vi "RemoteVI Send Origin.vi"(0 "clients":T1(array[cluster]), 5 "origin":cluster{"x":i32, "y":i32}, 7 "origin sent":cluster{"x":i32, "y":i32}) -> (4 "clients out":T1(array[cluster]), 6 "origin sent out":cluster{"x":i32, "y":i32})   [LabVIEW 2020, in "RemoteVI.lvlib"]
doc: "Tells every client where the panel area now starts inside the frame, when that changed: if origin differs from origin sent (the origin the clients were last told - new clients get the current one with their greeting), the text message origin x y (RemoteVI Origin Message.vi) is written to every client that is not closed (RemoteVI Write To Clients.vi, 500 ms per client; a failed write marks the client closed) and origin sent out becomes origin. Otherwise nothing is written."
uses:
  RemoteVI.lvlib
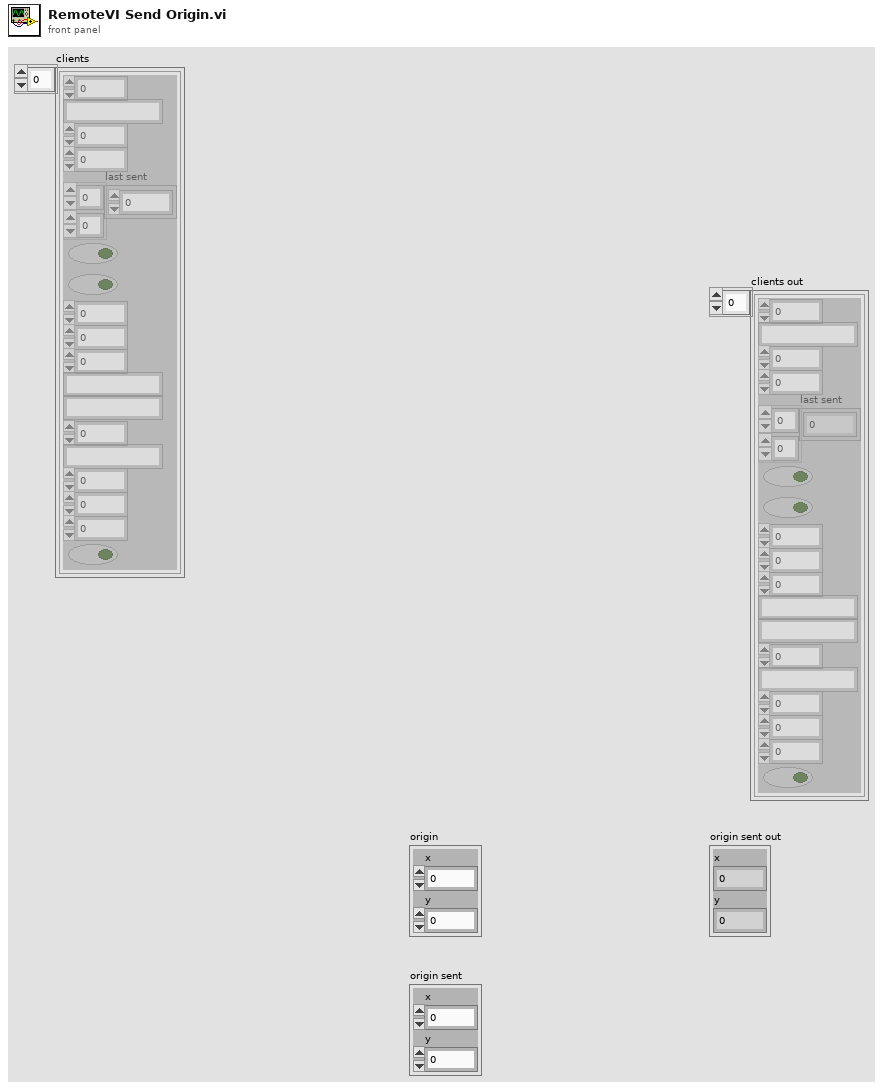
[diagram p1: front panel]
types:
  T1 = cluster{"connection":u32, "rx buffer":string, "seq":u32, "acked":u32, "last sent":u32[][], "tracking":bool, "closed":bool, "mods":u8, "mods set":u8, "popup since":u32, "windows sent":string, "window frames":cluster{"id":u64, "pixels":u32[][]}[], "key window":u64, "address":string, "since":dbl, "last input":dbl, "bytes":dbl, "view only":bool}[]
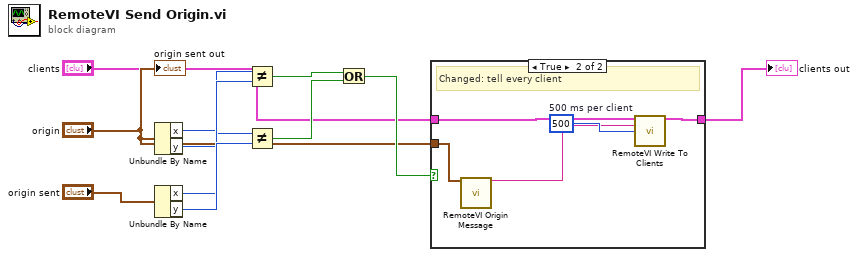
[diagram p0: block diagram]
diagram:
  n1 = Unbundle By Name("origin") -> ("x"=w4:i32, "y"=w5:i32)
  n2 = Unbundle By Name("origin sent") -> ("x"=w6:i32, "y"=w7:i32)
  n3 = Not Equal?(x=w4, y=w6) -> (x != y?=w8:bool)
  n4 = Not Equal?(x=w5, y=w7) -> (x != y?=w9:bool)
  n5 = Or(x=w8, y=w9) -> (x .or. y?=w10:bool)
  n6 = case shown="True" w10 {
    tunnel: "clients" -> [w12 w13]
    tunnel: "origin" -> [_ w14]
    tunnel: [w12 w17] -> w11
    frame False {
    }
    frame True {
      w16 = 500  # 500 ms per client
      # "Changed: tell every client"
      n7 = call "RemoteVI Origin Message.vi"("origin"=w14) -> ("frame"=w15:string)  [unwired: 14 in]
      n8 = call "RemoteVI Write To Clients.vi"("clients"=w13, "data"=w15, "timeout ms"=w16) -> ("clients out"=w17:T1)  [unwired: 12 in]
    }
  }
  "clients out" <- w11
  "origin sent out" <- "origin"
